vi "Test -- INI Creation.vi"() -> ()   [LabVIEW 2013]
uses:
  source/Manager.Text.INI/ConfigManager.Text.INI.lvclass
  source/Manager/Decompose KVPs.vi
  source/Manager/Write.vi
  source/Manager/ConfigManager.lvclass
  source/Manager.Text/ConfigManager.Text.lvclass
panel:
  in  "read-only?":bool
  out "Config":T1={"String"="test", "Numeric"=3.14159, "Boolean"=TRUE}
  out "text":string
  out "error out":errorcluster
  out "filepath":path
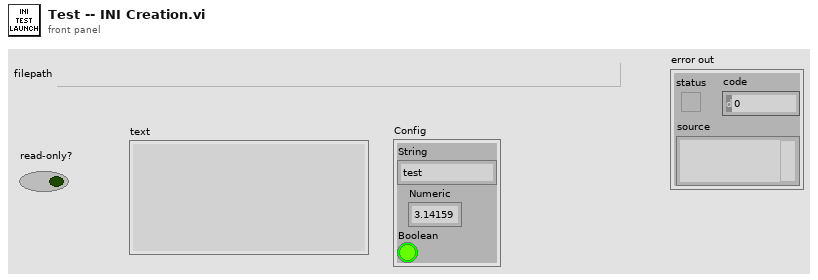
[diagram p1: front panel]
types:
  T1 = cluster{"String":string, "Numeric":dbl, "Boolean":bool}
  T2 = enum16{"open", "replace", "create", "open or create", "replace or create", "replace or create with confirmation"}
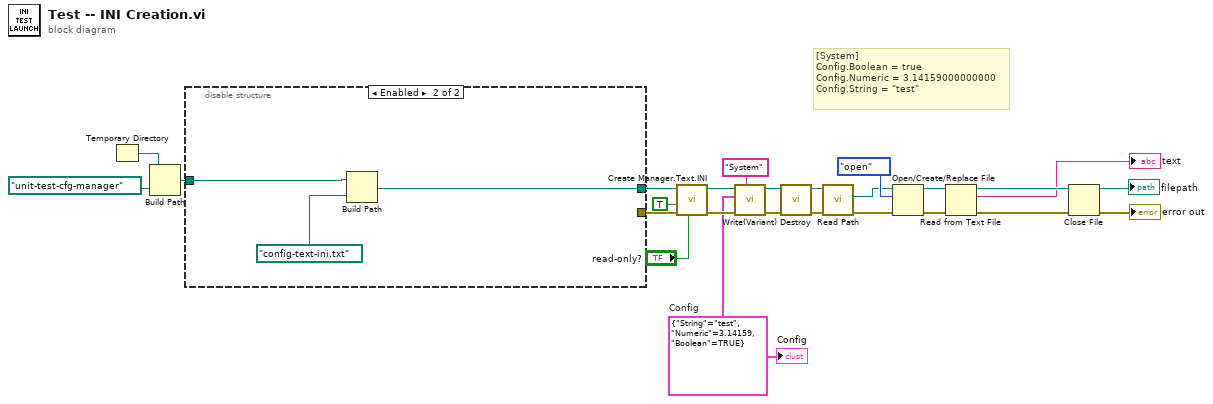
[diagram p0: block diagram]
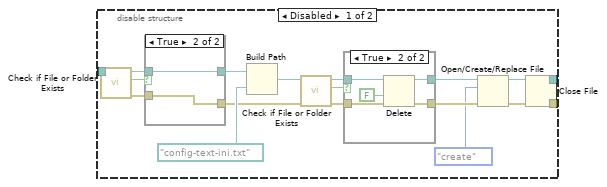
[diagram p2: hidden frame]
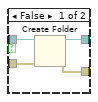
[diagram p4: hidden frame]
diagram:
  w18 = T1 {"String"="test", "Numeric"=3.14159, "Boolean"=TRUE}  # Config
  # "[System]\nConfig.Boolean = true\nConfig.Numeric = 3.14159000000000\nConfig.String = \"test\""
  n1 = Temporary Directory() -> (w23:path)
  n2 = Build Path(base path=w23, name or relative path=path "unit-test-cfg-manager") -> (appended path=w21:path)
  n3 = disable-structure shown="Enabled" {
    disable-tunnel: w21 -> [w42 w58]
    disable-tunnel: [w30 _] -> w14
    disable-tunnel: [w27 w56] -> w13
    frame Disabled {
      n4 = call <vilib>:"Check if File or Folder Exists.vi"("path"=w42) -> ("error out"=w37:errorcluster, "file or folder exists?"=w40:bool, "dup path"=w41:path)  [unwired: 8 in]
      n5 = case shown="True" w40 {
        tunnel: w41 -> [w53 w55]
        tunnel: [w52 w55] -> w39
        tunnel: w37 -> [w51 w54]
        tunnel: [w50 w54] -> w32
        frame False {
          n6 = Create Folder(path (use dialog)=w53, error in=w51) -> (created path=w52:path, error out=w50:errorcluster)  [unwired: 1 in, 1 out]
        }
        frame True {
        }
      }
      n7 = Build Path(base path=w39, name or relative path=path "config-text-ini.txt" ("filepath 2")) -> (appended path=w36:path)
      n8 = call <vilib>:"Check if File or Folder Exists.vi"("error in (no error)"=w32, "path"=w36) -> ("error out"=w34:errorcluster, "file or folder exists?"=w33:bool, "dup path"=w35:path)  [unwired: 7 in]
      n9 = case shown="True" w33 {
        tunnel: [w44 w48] -> w26
        tunnel: w35 -> [w44 w47]
        tunnel: w34 -> [w43 w46]
        tunnel: [w43 w45] -> w29
        frame False {
        }
        frame True {
          n10 = Delete(path (use dialog)=w47, confirm (F)=FALSE, error in=w46) -> (deleted path=w48:path, error out=w45:errorcluster)  [unwired: 2 in, 1 out]
        }
      }
      n11 = Open/Create/Replace File(file path (use dialog)=w26, error in=w29, operation (0:open)=T2."create") -> (refnum out=w28:refnum<file>, error out=w31:errorcluster)  [unwired: 3 in, 1 out]
      n12 = Close File(refnum=w28, error in=w31) -> (path=w27:path, error out=w30:errorcluster)
    }
    frame Enabled {
      n13 = Build Path(base path=w58, name or relative path=path "config-text-ini.txt" ("filepath 2")) -> (appended path=w56:path)
    }
  }
  n14 = call "Create Manager.Text.INI.vi"("read-only?"="read-only?", "error in (no error)"=w14, "Create if Non Existent? (T)"=TRUE, "filepath"=w13) -> ("error out"=w19:errorcluster, "ConfigManager.Text.INI out"=w20:refnum<class "ConfigManager.Text.INI.lvclass">)  [unwired: 5 in, 1 out]
  n15 = call "Write(Variant).vi"("Qualified Name"="System", "error in (no error)"=w19, "value"=w18, "ConfigManager in"=w20) -> ("error out"=w16:errorcluster, "ConfigManager out"=w17:refnum<class "ConfigManager.Text.INI.lvclass">)  [unwired: 5 in, 1 out]
  n16 = call-dynamic "Destroy.vi"("error in (no error)"=w16, "ConfigManager.Text in"=w17) -> ("error out"=w9:errorcluster, "ConfigManager.Text out"=w15:refnum<class "ConfigManager.Text.INI.lvclass">)  [unwired: 8 in]
  n17 = call "Read Path.vi"("ConfigManager.Text in"=w15) -> ("Path"=w11:path)  [unwired: 9 in, 1 out]
  n18 = Open/Create/Replace File(file path (use dialog)=w11, error in=w9, operation (0:open)=T2."open") -> (refnum out=w7:refnum<file>, error out=w5:errorcluster)  [unwired: 3 in, 1 out]
  n19 = Read from Text File(file (use dialog)=w7, error in=w5) -> (refnum out=w6:refnum<file>, text=→"text":string, error out=w4:errorcluster)  [unwired: 2 in, 1 out]
  n20 = Close File(refnum=w6, error in=w4) -> (path=→"filepath":path, error out=→"error out":errorcluster)
  "Config" <- w18
